vi "PicoScope2000ExampleBlock.vi"() -> ()   [LabVIEW 2010]
uses:
  shared/PicoBuffers.ctl
  shared/Buffer and Transfer Settings.ctl
  shared/Acquisition Settings.ctl
  PicoScope2000Lib/PicoScope2000AnalogChannelSettings.ctl
panel:
  in  "Trigger Settings":T1={"Trigger Enabled"=FALSE, "Trigger Source"=enum."Channel A", "Trigger Threshold (V)"=0.0, "Trigger Direction"=0, "Trigger Delay (%)"=0, "Auto Trigger Time (ms)"=1000} {"Trigger Direction" items=["Rising", "Falling"]; "Trigger Threshold (V)" format="%.3f"}
  in  "Channel B Settings":T2={"Enabled"=TRUE, "Coupling"=1, "Range"=6} {"Range" items=["20 mV"=1, "50 mV"=2, "100 mV"=3, "200 mV"=4, "500 mV"=5, "1 V"=6, "2 V"=7, "5 V"=8, "10 V"=9, "20 V"=10]; "Coupling" items=["AC", "DC"]}
  in  "Channel A Settings":T2={"Enabled"=TRUE, "Coupling"=1, "Range"=7} {"Range" items=["20 mV"=1, "50 mV"=2, "100 mV"=3, "200 mV"=4, "500 mV"=5, "1 V"=6, "2 V"=7, "5 V"=8, "10 V"=9, "20 V"=10]; "Coupling" items=["AC", "DC"]}
  out "Unit Info":T3={"Driver Version"="", "USB Version"="", "Hardware"="", "Variant"="", "Batch and Serial"="", "Cal Date"="", "Kernel Version"="0"}
  out "overflow":i16 format="%010b"
  in  "Apply Settings":bool
  out "error out":errorcluster
  in  "Data file":path=path "PicoScope2000ExampleBlock ChA Data"
  in  "Buffer and Transfer Settings":T4={"startIndex"=0, "Samples"=3968, "Down Sample Ratio"=1, "Down-Sample Mode"=0} {"Down-Sample Mode" items=["RAW none"=2147483648, "None"=0, "Aggregate"=1, "Decimate"=2, "Average"=4]; "Down Sample Ratio" step=1; "Samples" format="%_6p"}
  in  "Acquisition Settings":T5={"preTriggerSamples"=0, "postTriggerSamples"=3968, "timebase"=5} {"postTriggerSamples" format="%_6p"; "preTriggerSamples" format="%_6p"}
  out "Properties Panel":T6 {"Max Total Capture Time Available (sec)" format="%.3p"; "Sample Frequency" format="%.6p"; "Sample Rate" format="%.3p"; "Max Samples Available" format="%_6p"; "Total Capture Time (sec)" format="%.3p"}
  in  "stop":bool
  out "Analog Channels":T7(graph)
  in  "error in (no error)":errorcluster
  # "Bit 0 = ChA"
  # "Oversample control ->"
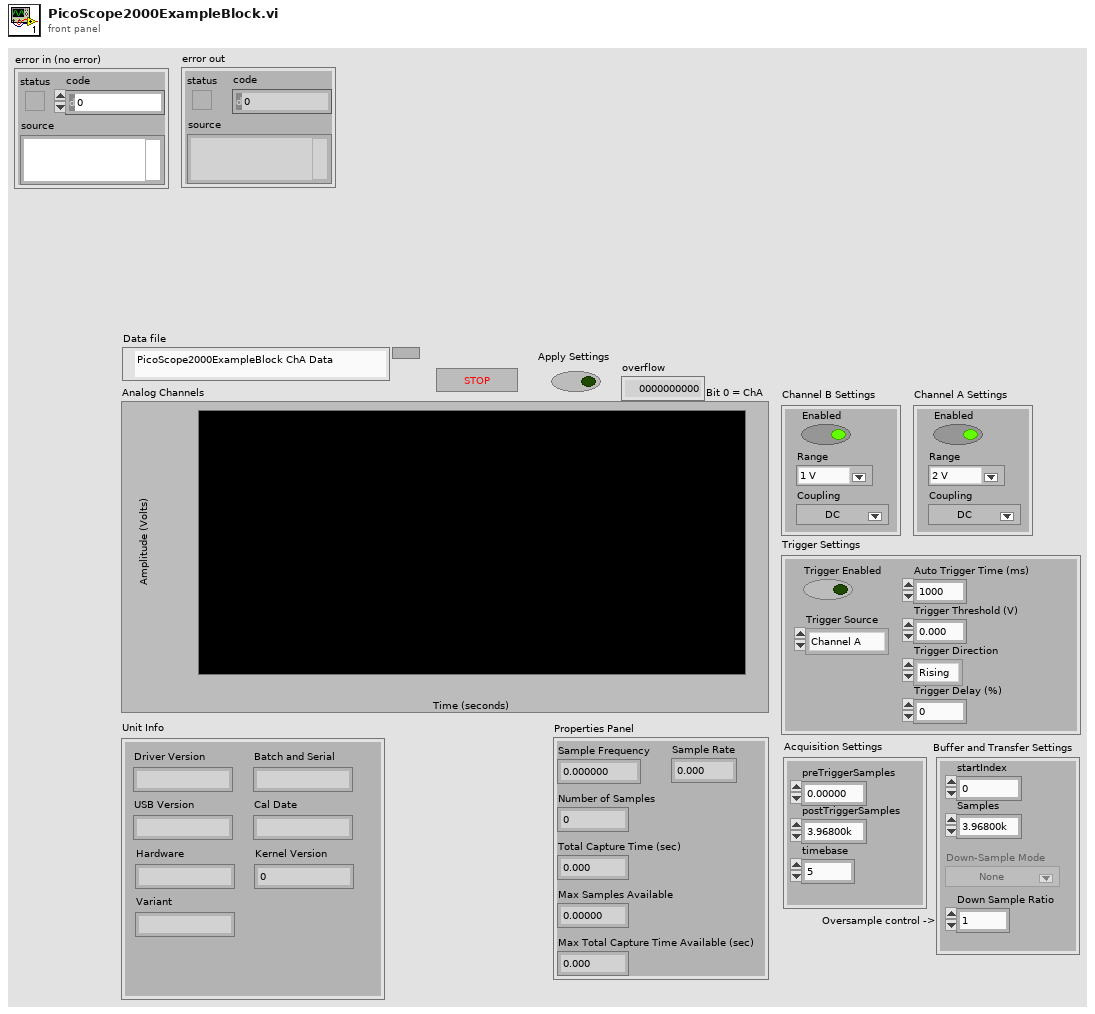
[diagram p1: front panel]
types:
  T1 = cluster{"Trigger Enabled":bool, "Trigger Source":enum16{"Channel A", "Channel B"}, "Trigger Threshold (V)":dbl, "Trigger Direction":i16, "Trigger Delay (%)":i16, "Auto Trigger Time (ms)":i16}
  T2 = typedef "PicoScope2000AnalogChannelSettings.ctl" = cluster{"Enabled":bool, "Coupling":i16, "Range":u16}
  T3 = cluster{"Driver Version":string, "USB Version":string, "Hardware":string, "Variant":string, "Batch and Serial":string, "Cal Date":string, "Kernel Version":string}
  T4 = typedef "Buffer and Transfer Settings.ctl" = cluster{"startIndex":u64, "Samples":u64, "Down Sample Ratio":u64, "Down-Sample Mode":u32}
  T5 = typedef "Acquisition Settings.ctl" = cluster{"preTriggerSamples":u64, "postTriggerSamples":u64, "timebase":u32}
  T6 = cluster{"Sample Frequency":dbl, "Sample Rate":dbl, "Max Samples Available":u64, "Number of Samples":u64, "Total Capture Time (sec) ":dbl, "Max Total Capture Time Available (sec)":dbl}
  T7 = cluster{i32, "Down Sample Ratio":u64, "Data":dbl[]}[]
  T8 = typedef "PicoBuffers.ctl" = cluster{"Max Buffer Pointers":u64[][][], "Min Buffer Pointers":u64[][][], "StreamingDataInfo":cluster{"Channel":u32, "Down-Sample Mode":u32, "PICO_DATA_TYPE":enum32{"PICO_INT8_T", "PICO_INT16_T", "PICO_INT32_T", "PICO_UINT32_T", "PICO_INT64_T", ""}, "Samples":i32, "bufferIndex":u64, "startIndex":i32, "overflow":i16}[][]}
  T9 = enum16{"open", "open or create", "create or replace", "create", "open (read-only)"}
  T10 = cluster{"Sample Frequency":sgl, "Sample Rate":sgl, "Max Samples Available":i32, "Number of Samples":u32, "Total Capture Time (sec) ":sgl, "Max Total Capture Time Available (sec)":sgl}
  T11 = cluster{"Channel A Buffer":i16[], "Channel B Buffer":i16[], "Channel C Buffer":i16[], "Channel D Buffer":i16[], "Channel E Buffer":i16[], "Channel F Buffer":i16[], "Channel G Buffer":i16[], "Channel H Buffer":i16[], "Port 0 Buffer":i16[], "Port 1 Buffer":i16[]}[]
  T12 = cluster{"Channel A Buffer":i16[], "Channel B Buffer":i16[], "Channel C Buffer":i16[], "Channel D Buffer":i16[], "Channel E Buffer":i16[], "Channel F Buffer":i16[], "Channel G Buffer":i16[], "Channel H Buffer":i16[], "Port 0 Buffer":i16[], "Port 1 Buffer":i16[]}
  T13 = cluster{i32, "Down Sample Ratio":u64, "Data":dbl[]}
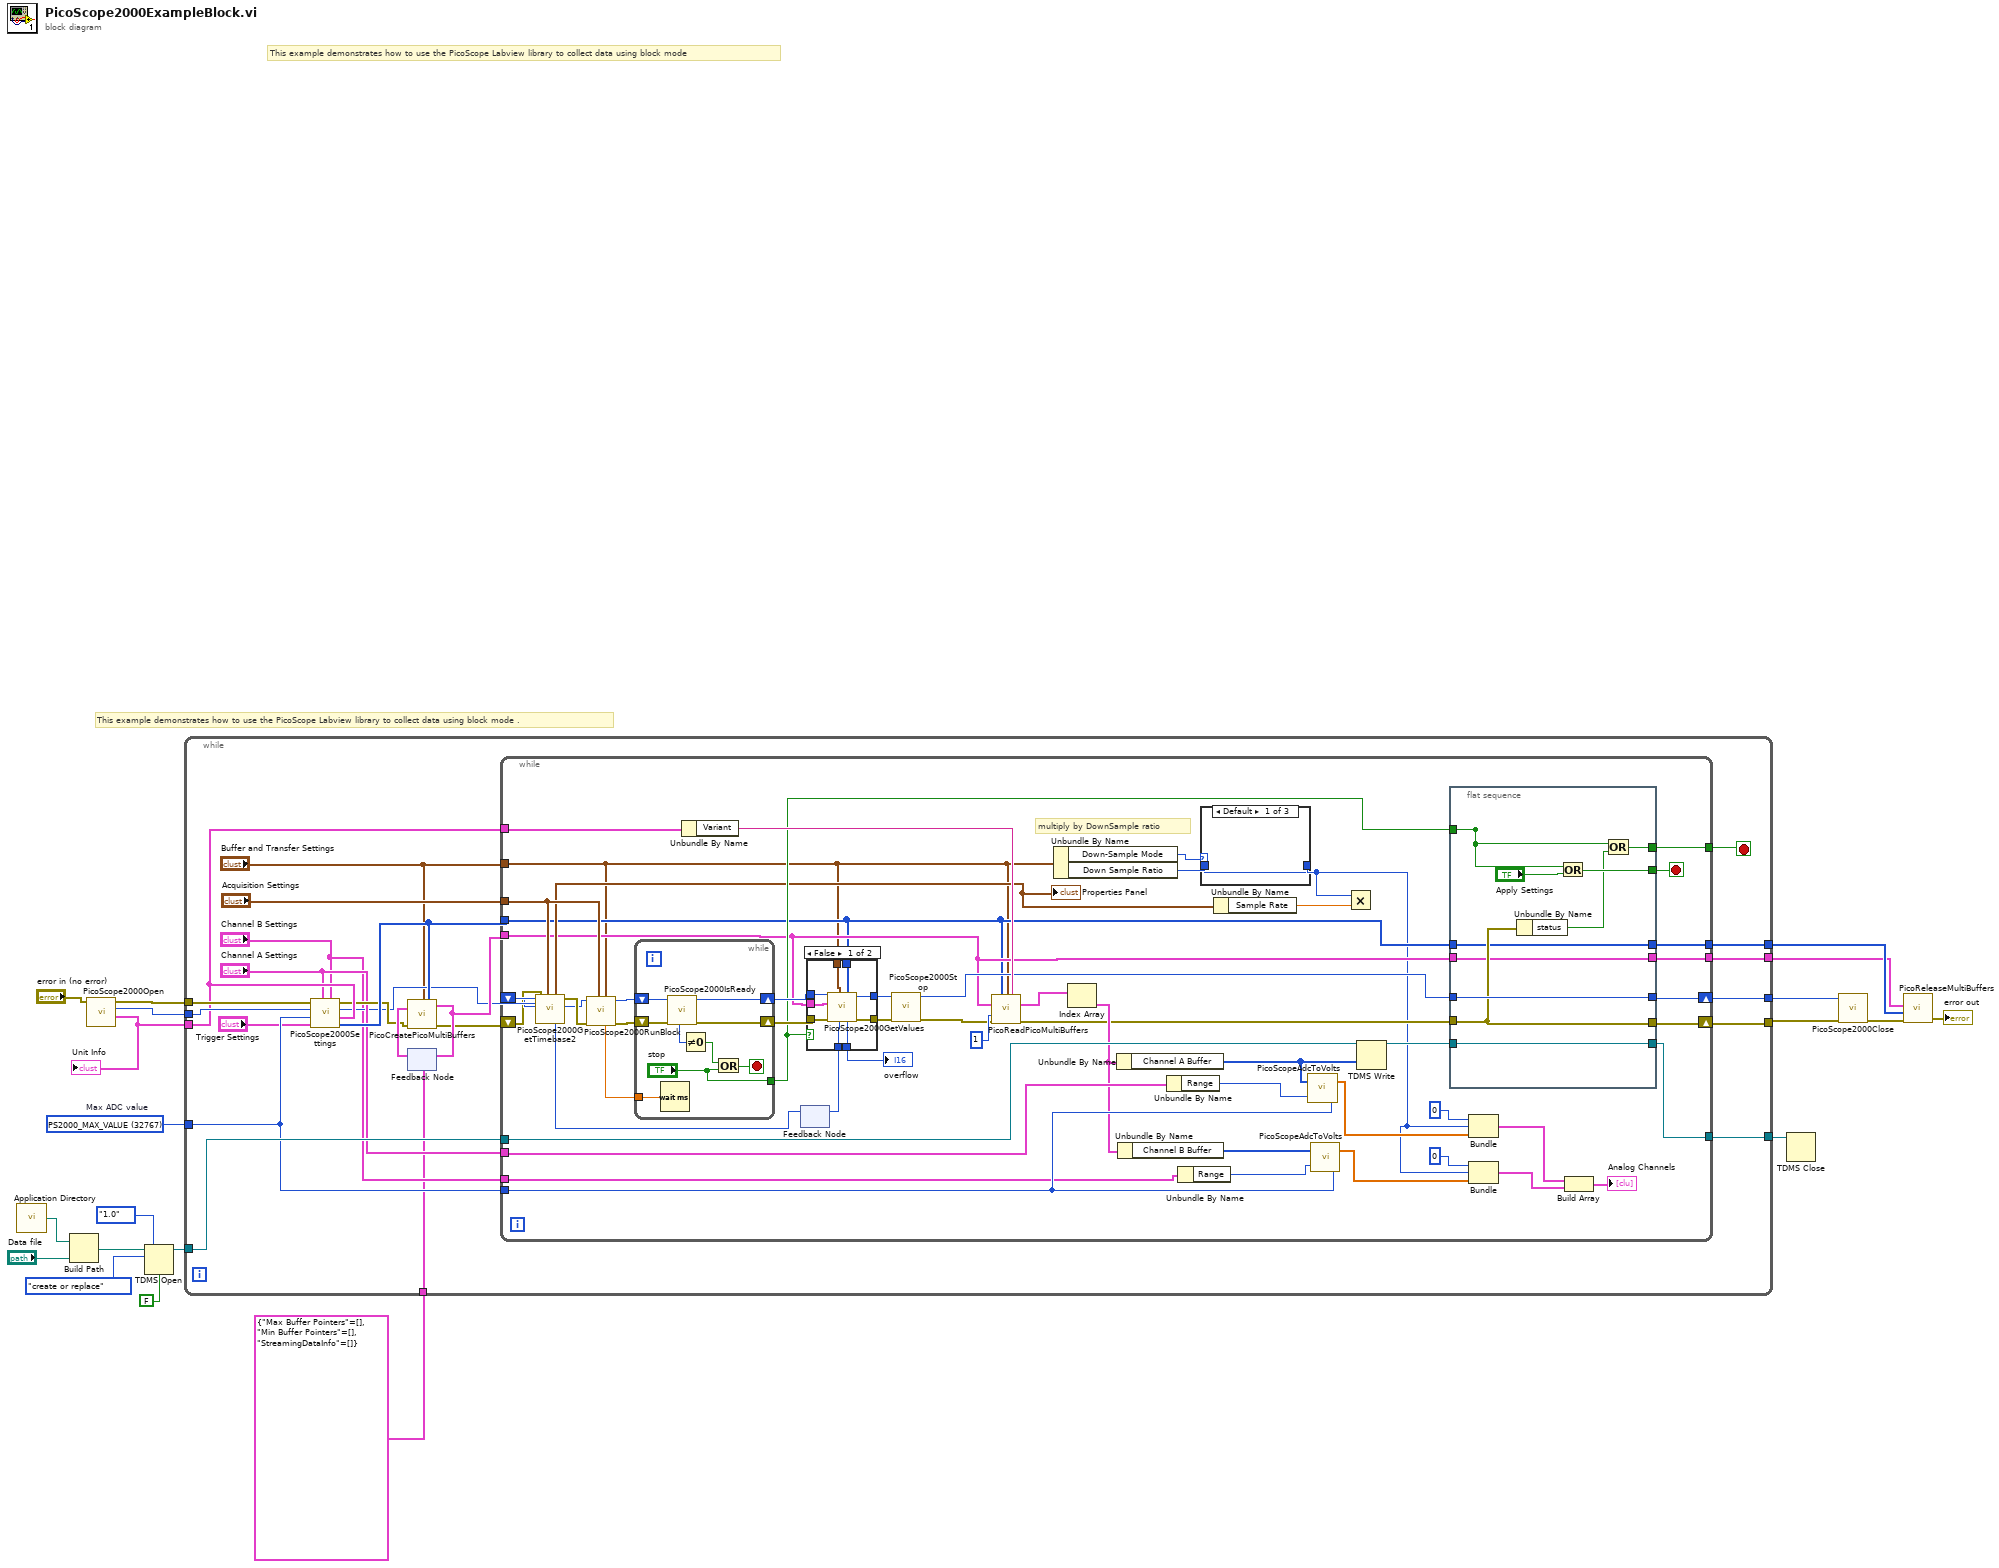
[diagram p0: block diagram]
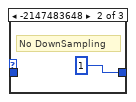
[diagram p3: hidden frame]
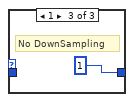
[diagram p4: hidden frame]
diagram:
  w1 = i16 32767 items=["PS2000_MAX_VALUE"=32767]  # Max ADC value
  # "This example demonstrates how to use the PicoScope Labview library to collect data using block mode ."
  # "This example demonstrates how to use the PicoScope Labview library to collect data using block mode"
  n1 = call <vilib>:"Application Directory.vi"() -> ("Application Directory"=w13:path)
  n2 = Build Path(base path=w13, name or relative path="Data file") -> (appended path=w14:path)
  n3 = call "PicoScope2000Open.vi"("error in (no error)"="error in (no error)") -> ("Unit Info"=w5:T3, "handle"=w6:i16, "error out"=w7:errorcluster)  [unwired: 6 in]
  "Unit Info" <- w5
  n4 = TDMS Open(6:FALSE ("disable buffering? (T)"), 7:enum16{"1.0", "2.0"}."1.0" ("file format version (2.0)"), 10:T9."create or replace" ("operation (0:open)"), 11:w14) -> (3:w11:refnum<k34>)  [unwired: 2 in, 1 out]
  n5 = while {
    tunnel: w6 -> [w40]
    tunnel: w1 -> [w34]
    tunnel: [w22] -> w20
    tunnel: [w23] -> w19
    tunnel: [w37] -> w12
    tunnel: w11 -> [w41]
    tunnel: w5 -> [w32]
    tunnel: w7 -> [w39]
    tunnel: [w38] -> w3
    tunnel: [w35] -> w4
    tunnel: T8 {"Max Buffer Pointers"=[], "Min Buffer Pointers"=[], "StreamingDataInfo"=[]} ("Data Pointers") -> [w21]
    stop <- w36 stop-if-true
    n6 = call "PicoScope2000Settings.vi"("Unit Info"=w32, "Channel B Settings"="Channel B Settings", "Channel A Settings"="Channel A Settings", "Trigger Settings"="Trigger Settings", "Max ADC value"=w34, "handle in"=w40, "error in"=w39) -> ("Enabled Array"=w33:i16[], "handle out"=w28:i16, "error out"=w31:errorcluster)
    n7 = feedback #1(w21) -> (w43:T8)
    n8 = call "PicoCreatePicoMultiBuffers.vi"("Buffer and Transfer Settings"="Buffer and Transfer Settings", "enabled array"=w33, "Data Pointers In"=w43, "error in (no error)"=w31) -> ("Data Pointers"=w42:T8, "error out"=w29:errorcluster)  [unwired: 10 in]
    n9 = feedback-in #1(w42) -> ()
    n10 = while {
      tunnel: w42 -> [w49]
      tunnel: "Buffer and Transfer Settings" -> [w44]
      tunnel: w33 -> [w46]
      tunnel: "Channel A Settings" -> [w92]
      tunnel: "Acquisition Settings" -> [w57]
      tunnel: w34 -> [w91]
      tunnel: w32 -> [w88]
      tunnel: [w70] -> w36
      shift-right: [w74] -> w38
      shift-left: w29 -> [w58]
      shift-right: [w68] -> w35
      shift-left: w28 -> [w59]
      tunnel: w41 -> [w98]
      tunnel: [w72] -> w37
      tunnel: "Channel B Settings" -> [w62]
      tunnel: [w48] -> w23
      tunnel: [w47] -> w22
      stop <- w69 stop-if-true
      # "multiply by DownSample ratio"
      n11 = Unbundle By Name(w88) -> ("Variant"=w89:string)
      n12 = feedback #2() -> (w55:u64)  [unwired: 1 in]
      n13 = call "PicoScope2000GetTimebase2.vi"("Number of Samples"=w55, "Acquisition Settings"=w57, "handle in"=w59, "error in (no error)"=w58) -> ("handle out"=w60:i16, "error out"=w61:errorcluster, "Properties Panel"=w54:T10)  [unwired: 5 in]
      "Properties Panel" <- w54
      n14 = call "PicoScope2000RunBlock.vi"("Buffer and Transfer Settings"=w44, "Acquisition Settings"=w57, "error in (no error)"=w61, "handle in"=w60) -> ("error out"=w94:errorcluster, "handle out"=w93:i16, "timeIndisposedMs"=w86:dbl)  [unwired: 4 in, 1 out]
      n15 = while {
        shift-right: [w127] -> w66
        shift-left: w94 -> [w128]
        shift-right: [w126] -> w67
        shift-left: w93 -> [w125]
        tunnel: ["stop"] -> w65
        tunnel: w86 -> [w120]
        stop <- w122 stop-if-true
        n16 = Wait (ms)(milliseconds to wait=w120) -> ()  [unwired: 1 out]
        n17 = call "PicoScope2000IsReady.vi"("error in (no error)"=w128, "handle in"=w125) -> ("error out"=w127:errorcluster, "handle out"=w126:i16, "ready"=w124:i16)  [unwired: 7 in]
        n18 = Not Equal To 0?(x=w124) -> (x != 0?=w123:bool)
        n19 = Or(x=w123, y="stop") -> (x .or. y?=w122:bool)
      }
      n20 = case shown="False" w65 {
        tunnel: w66 -> [w107 w108]
        tunnel: w67 -> [w106 w109]
        tunnel: [w105 w109] -> w53
        tunnel: [w104 w108] -> w52
        tunnel: [w103 _] -> w64
        tunnel: [w102 _] -> w56
        tunnel: w46 -> [w101 _]
        tunnel: w49 -> [w100 _]
        tunnel: w44 -> [w99 _]
        frame False {
          n21 = call "PicoScope2000GetValues.vi"("enabled array"=w101, "Buffer and Transfer Settings"=w99, "error in (no error)"=w107, "Data Pointers In"=w100, "handle in"=w106) -> ("error out"=w104:errorcluster, "handle out"=w105:i16, "overflow"=w103:i16, "noOfSamples"=w102:u64)  [unwired: 3 in]
        }
        frame True {
        }
      }
      "overflow" <- w64
      n22 = feedback-in #2(w56) -> ()
      n23 = call "PicoScope2000Stop.vi"("error in (no error)"=w52, "handle in"=w53) -> ("error out"=w51:errorcluster, "handle out"=w50:i16)  [unwired: 8 in]
      n24 = call "PicoReadPicoMultiBuffers.vi"("enabled array"=w46, "Buffer and Transfer Settings"=w44, "Variant"=w89, "Data Pointers"=w49, "No of Buffers"=1, "error in (no error)"=w51) -> ("MultiBuffers (Max or non-aggregated)"=w97:T11, "error out"=w71:errorcluster)  [unwired: 7 in, 1 out]
      n25 = Unbundle By Name(w44) -> ("Down-Sample Mode"=w95:u32, "Down Sample Ratio"=w96:u64)
      n26 = Index Array(array=w97) -> (element=w75:T12)  [unwired: 1 in]
      n27 = Unbundle By Name(w75) -> ("Channel A Buffer"=w76:i16[])
      n28 = Unbundle By Name(w75) -> ("Channel B Buffer"=w82:i16[])
      n29 = Unbundle By Name(w92) -> ("Range"=w84:u16)
      n30 = Unbundle By Name(w62) -> ("Range"=w63:u16)
      n31 = case shown="Default" w95 {
        tunnel: [w129 u64 1 ("Down Sample Ratio") u64 1 ("Down Sample Ratio")] -> w45
        tunnel: w96 -> [w129 _ _]
        frame Default {
        }
        frame -2147483648 {
          # "No DownSampling"
        }
        frame 1 {
          # "No DownSampling"
        }
      }
      n32 = Unbundle By Name(w54) -> ("Sample Rate"=w90:sgl)
      n33 = call "PicoScopeAdcToVolts.vi"("Max_adc"=w91, "Range Index"=w84, "Data"=w76) -> ("Data"=w77:dbl[])
      n34 = call "PicoScopeAdcToVolts.vi"("Max_adc"=w91, "Range Index"=w63, "Data"=w82) -> ("Data"=w81:dbl[])
      n35 = Multiply(x=w45, y=w90) -> ()  [unwired: 1 out]
      n36 = TDMS Write(0:w98, 9:w76) -> (4:w73:refnum<k34>)  [unwired: 4 in, 3 out]
      n37 = flat-sequence {
        tunnel: [w119] -> w69
        tunnel: [w112] -> _
        tunnel: [w116] -> w70
        tunnel: w50 -> [w115]
        tunnel: [w115] -> w68
        tunnel: w71 -> [w114]
        tunnel: [w114] -> w74
        tunnel: [w113] -> w72
        tunnel: w73 -> [w113]
        tunnel: w65 -> [w112]
        tunnel: w49 -> [w111]
        tunnel: [w111] -> w48
        tunnel: [w110] -> w47
        tunnel: w46 -> [w110]
        frame #0 {
          n38 = Unbundle By Name(w114) -> ("status"=w117:bool)
          n39 = Or(x=w112, y="Apply Settings") -> (x .or. y?=w119:bool)
          n40 = Or(x=w112, y=w117) -> (x .or. y?=w116:bool)
        }
      }
      n41 = Bundle(0, "Down Sample Ratio"=w45, "Data"=w77) -> (w80:T13)  [unwired: 1 in]
      n42 = Bundle(0, "Down Sample Ratio"=w45, "Data"=w81) -> (w79:T13)  [unwired: 1 in]
      n43 = Build Array(w80, w79) -> (→"Analog Channels":T7)
    }
  }
  n44 = TDMS Close(11:w12) -> ()  [unwired: 1 in, 2 out]
  n45 = call "PicoScope2000Close.vi"("error in"=w3, "handle"=w4) -> ("error out"=w8:errorcluster)  [unwired: 4 in, 1 out]
  n46 = call "PicoReleaseMultiBuffers.vi"("error in (no error)"=w8, "Enabled array"=w20, "Data Pointers"=w19) -> ("error out"=→"error out":errorcluster)  [unwired: 8 in]
